vi "main.vi"() -> ()   [LabVIEW 2026]
uses:
  <vilib>/Instr/_visa.llb/VISA Configure Serial Port (Instr).vi
panel:
  out "보내는 패킷":string
  out "상태명령":string
  out "상태바뀜":bool
  out "하트비트 보냄":bool
  out "하트비트 패킷":string
  out "서보패킷":string
  in  "서보 보내기":bool
  in  "각도":u8
  in  "채널":u8
  in  "COM 포트":refnum<visa-resource-name>
  in  "박수 보내기":bool
  out "현재 상태":enum8{"대기", "트리거감지", "반응", "탐색이동", "회피", "복귀"}(ring)
  in  "Boolean":bool
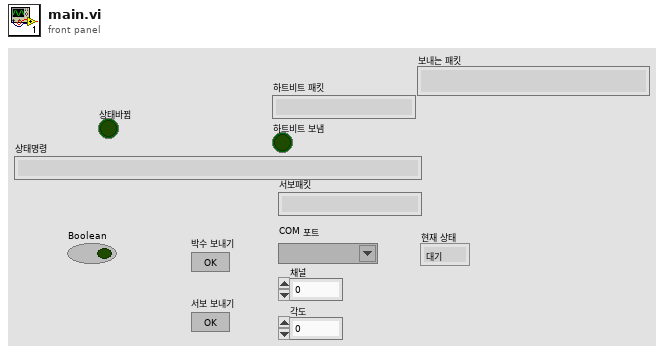
[diagram p1: front panel]
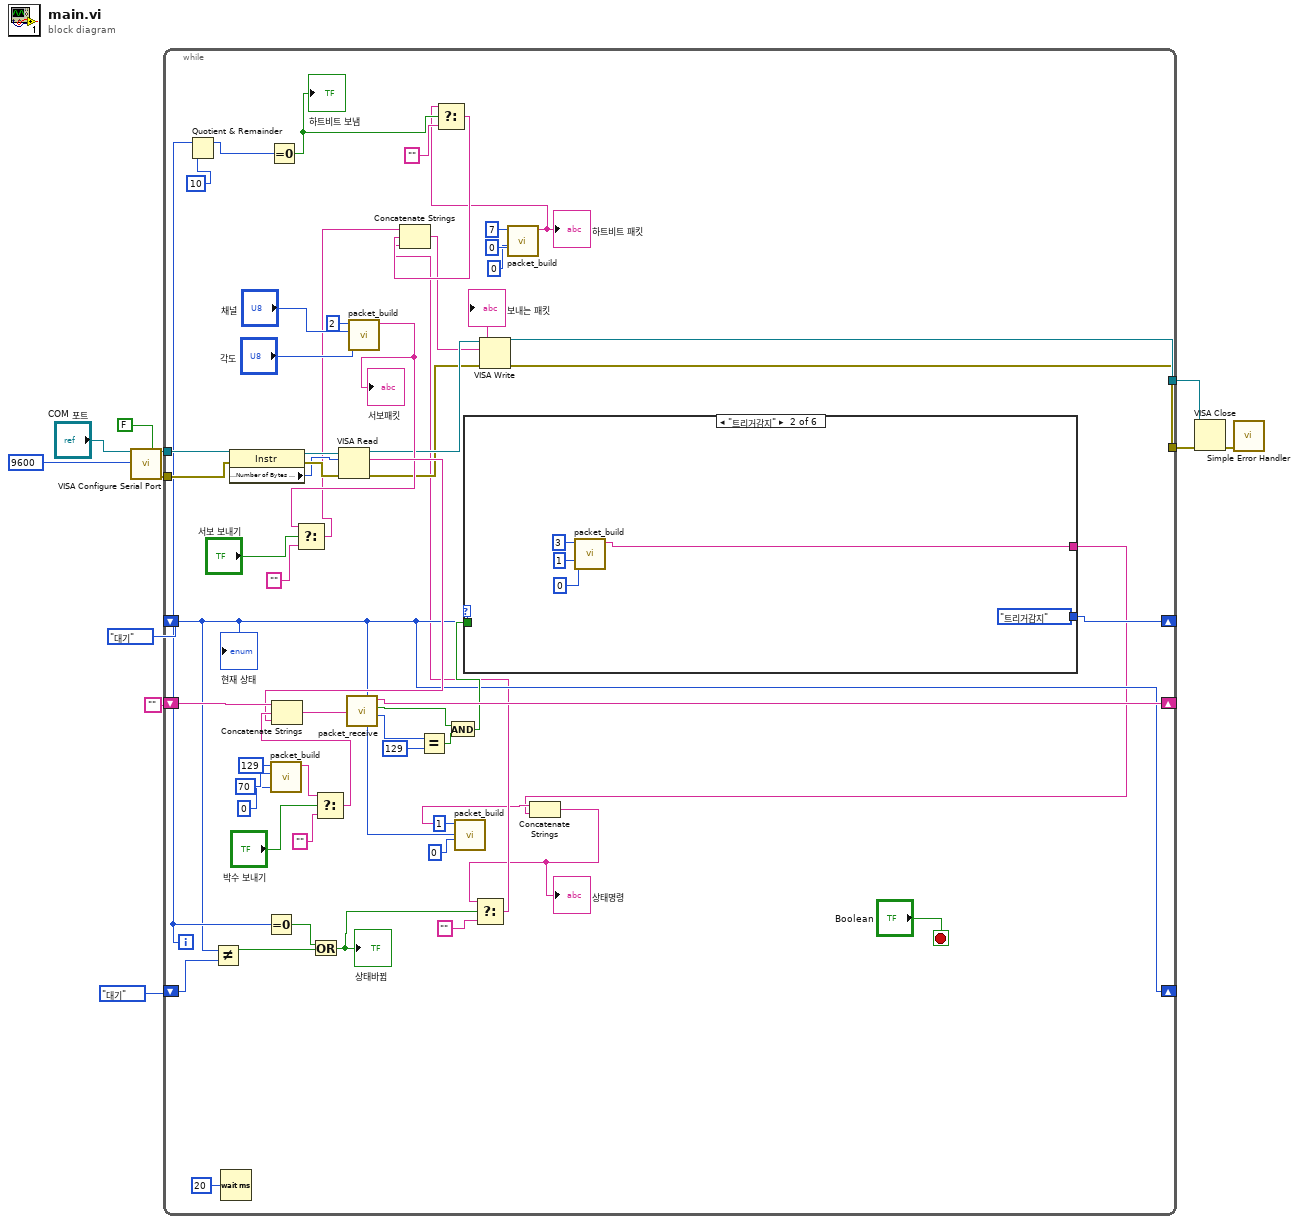
[diagram p0: block diagram]
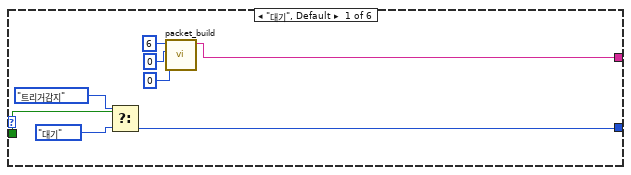
[diagram p2: hidden frame]
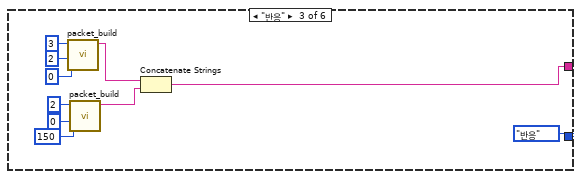
[diagram p3: hidden frame]
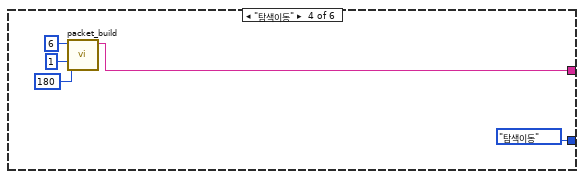
[diagram p4: hidden frame]
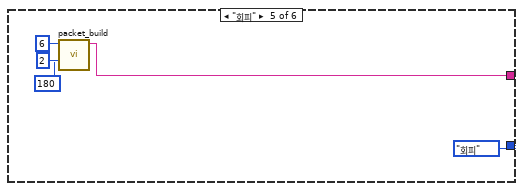
[diagram p5: hidden frame]
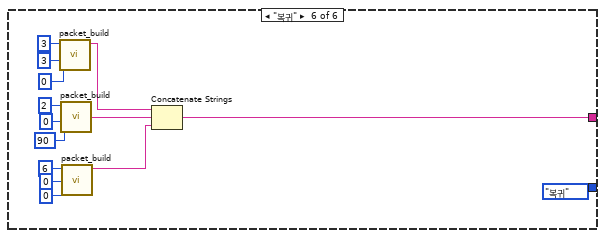
[diagram p6: hidden frame]
diagram:
  n1 = call-poly "VISA Configure Serial Port"("VISA resource name"="COM 포트", "Enable Termination\nChar (T)"=FALSE ("Enable Termination\nChar (T)"), "baud rate (9600)"=u32 9600) -> ("VISA resource name out"=w6:refnum<visa-resource-name>, "error out"=w5:errorcluster)  [unwired: 11 in]
  n2 = while {
    shift-right: [w68] -> _
    shift-left: enum8{"대기", "트리거감지", "반응", "탐색이동", "회피", "복귀"}."대기" -> [w18]
    shift-right: [w57] -> _
    shift-left: "" -> [w60]
    tunnel: w6 -> [w51]
    tunnel: w5 -> [w50]
    tunnel: [w37] -> w4
    tunnel: [w36] -> w3
    shift-right: [w18] -> _
    shift-left: enum8{"대기", "트리거감지", "반응", "탐색이동", "회피", "복귀"}."대기" -> [w25]
    i -> [w24]
    stop <- "Boolean" stop-if-true
    n3 = Quotient & Remainder(x=w24, y=10) -> (x-y*floor(x/y)=w26:i32)  [unwired: 1 out]
    n4 = Not Equal?(x=w18, y=w25) -> (x != y?=w22:bool)
    n5 = Wait (ms)(milliseconds to wait=u32 20) -> ()  [unwired: 1 out]
    n6 = property class="Instr"(reference=w51, error in=w50) -> (reference out=w49:refnum<visa-resource-name>, error out=w48:errorcluster, "Serial Settings:Number of Bytes at Serial Port"=w47:u32)
    n7 = Equal To 0?(x=w24) -> (x = 0?=w23:bool)
    n8 = Equal To 0?(x=w26) -> (x = 0?=w31:bool)
    "하트비트 보냄" <- w31
    n9 = call "packet_build.vi"("D2"=u8 0, "D1"=u8 70, "CMD"=u8 129) -> ("packet"=w61:string)  [unwired: 8 in]
    n10 = Or(x=w23, y=w22) -> (x .or. y?=w19:bool)
    "상태바뀜" <- w19
    n11 = Select(t=w61, s="박수 보내기", f="") -> (s? t:f=w59:string)
    n12 = VISA Read(VISA resource name=w49, byte count=w47, error in (no error)=w48) -> (VISA resource name out=w39:refnum<visa-resource-name>, read buffer=w46:string, error out=w38:errorcluster)  [unwired: 1 out]
    n13 = Concatenate Strings(w60, w59, w46) -> (w58:string)
    n14 = call "packet_receive.vi"("버퍼 in"=w58) -> ("CMD"=w56:u8, "유효"=w54:bool, "버퍼 out"=w57:string)  [unwired: 6 in, 2 out]
    n15 = call "packet_build.vi"("D2"="각도", "D1"="채널", "CMD"=u8 2) -> ("packet"=w42:string)  [unwired: 8 in]
    "서보패킷" <- w42
    n16 = Select(t=w42, s="서보 보내기", f="") -> (s? t:f=w29:string)
    n17 = Equal?(x=w56, y=u8 129) -> (x = y?=w53:bool)
    n18 = And(x=w54, y=w53) -> (x .and. y?=w52:bool)
    n19 = call "packet_build.vi"("D2"=u8 0, "D1"=w18, "CMD"=u8 1) -> ("packet"=w15:string)  [unwired: 8 in]
    n20 = case shown="\"트리거감지\"" w18 {
      tunnel: [w74 enum8{"대기", "트리거감지", "반응", "탐색이동", "회피", "복귀"}."트리거감지" enum8{"대기", "트리거감지", "반응", "탐색이동", "회피", "복귀"}."반응" enum8{"대기", "트리거감지", "반응", "탐색이동", "회피", "복귀"}."탐색이동" enum8{"대기", "트리거감지", "반응", "탐색이동", "회피", "복귀"}."회피" enum8{"대기", "트리거감지", "반응", "탐색이동", "회피", "복귀"}."복귀"] -> w68
      tunnel: w52 -> [w76 _ _ _ _ _]
      tunnel: [w70 w78 w83 w93 w98 w103] -> w13
      frame "대기", Default {
        n21 = Select(t=enum8{"대기", "트리거감지", "반응", "탐색이동", "회피", "복귀"}."트리거감지", s=w76, f=enum8{"대기", "트리거감지", "반응", "탐색이동", "회피", "복귀"}."대기") -> (s? t:f=w74:enum8{"대기", "트리거감지", "반응", "탐색이동", "회피", "복귀"})
        n22 = call "packet_build.vi"("D2"=u8 0, "D1"=u8 0, "CMD"=u8 6) -> ("packet"=w70:string)  [unwired: 8 in]
      }
      frame "트리거감지" {
        n23 = call "packet_build.vi"("D2"=u8 0, "D1"=u8 1, "CMD"=u8 3) -> ("packet"=w78:string)  [unwired: 8 in]
      }
      frame "반응" {
        n24 = call "packet_build.vi"("D2"=u8 0, "D1"=u8 2, "CMD"=u8 3) -> ("packet"=w85:string)  [unwired: 8 in]
        n25 = call "packet_build.vi"("D2"=u8 150, "D1"=u8 0, "CMD"=u8 2) -> ("packet"=w84:string)  [unwired: 8 in]
        n26 = Concatenate Strings(w85, w84) -> (w83:string)
      }
      frame "탐색이동" {
        n27 = call "packet_build.vi"("D2"=u8 180, "D1"=u8 1, "CMD"=u8 6) -> ("packet"=w93:string)  [unwired: 8 in]
      }
      frame "회피" {
        n28 = call "packet_build.vi"("D2"=u8 180, "D1"=u8 2, "CMD"=u8 6) -> ("packet"=w98:string)  [unwired: 8 in]
      }
      frame "복귀" {
        n29 = call "packet_build.vi"("D2"=u8 0, "D1"=u8 3, "CMD"=u8 3) -> ("packet"=w106:string)  [unwired: 8 in]
        n30 = call "packet_build.vi"("D2"=u8 90, "D1"=u8 0, "CMD"=u8 2) -> ("packet"=w105:string)  [unwired: 8 in]
        n31 = call "packet_build.vi"("D2"=u8 0, "D1"=u8 0, "CMD"=u8 6) -> ("packet"=w104:string)  [unwired: 8 in]
        n32 = Concatenate Strings(w106, w105, w104) -> (w103:string)
      }
    }
    n33 = call "packet_build.vi"("D2"=u8 0, "D1"=u8 0, "CMD"=u8 7) -> ("packet"=w12:string)  [unwired: 8 in]
    "하트비트 패킷" <- w12
    n34 = Select(t=w12, s=w31, f="") -> (s? t:f=w28:string)
    n35 = Concatenate Strings(w15, w13) -> (w14:string)
    "상태명령" <- w14
    n36 = Select(t=w14, s=w19, f="") -> (s? t:f=w16:string)
    n37 = Concatenate Strings(w29, w28, w16) -> (w27:string)
    "보내는 패킷" <- w27
    n38 = VISA Write(VISA resource name=w39, write buffer=w27, error in (no error)=w38) -> (VISA resource name out=w37:refnum<visa-resource-name>, error out=w36:errorcluster)  [unwired: 1 out]
    "현재 상태" <- w18
  }
  n39 = VISA Close(VISA resource name=w4, error in (no error)=w3) -> (error out=w2:errorcluster)
  n40 = call <vilib>:"Simple Error Handler.vi"("error in (no error)"=w2) -> ()  [unwired: 4 in, 5 out]
